vi "Stop.vi"(8 "error in (no error)":errorcluster, 11 "XNET_CAN_RW in":refnum<class "XNET CAN RW.lvclass">) -> (0 "error out":errorcluster, 3 "XNET_CAN_RW out":refnum<class "XNET CAN RW.lvclass">)   [LabVIEW 2021, in "XNET CAN RW.lvclass"]
uses:
  XNET CAN RW.lvclass
  XNET CAN RW.lvclass/XNET CAN RW.ctl
  <vilib>/Utility/error.llb/Clear Errors.vi
  Utilities/Add Error.vi
  <vilib>/xnet/xnet.llb/XNET Wait (Transmit Complete).vi
  Utilities/Add Error Core.vi
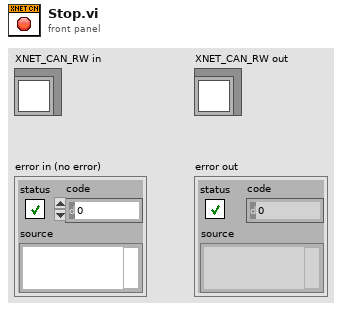
[diagram p1: front panel]
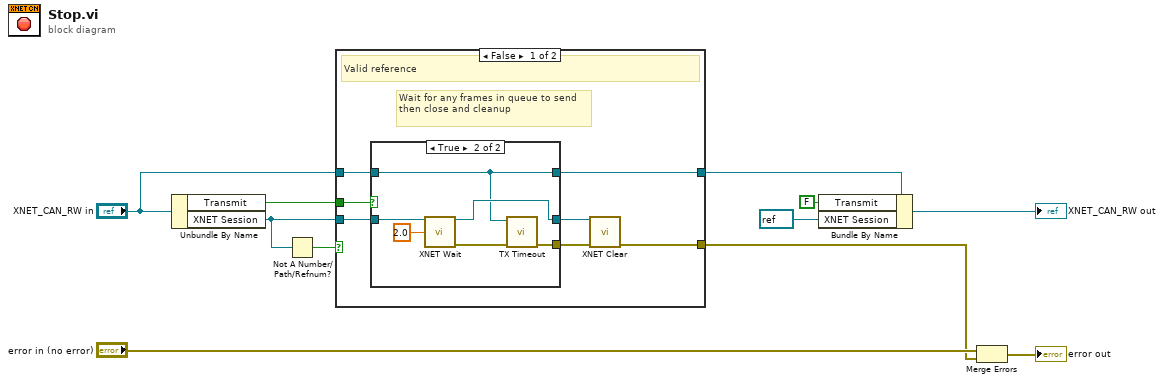
[diagram p0: block diagram]
diagram:
  n1 = Unbundle By Name("XNET_CAN_RW in") -> ("Transmit"=w4:bool, "XNET Session"=w6:refnum<k21>)
  n2 = Not A Number/Path/Refnum?(number/path/refnum=w6) -> (NaN/Path/Refnum?=w7:bool)
  n3 = case shown="False" w7 {
    tunnel: w6 -> [w18 _]
    tunnel: [w17 _] -> w9
    tunnel: w4 -> [w14 _]
    tunnel: "XNET_CAN_RW in" -> [w13 w27]
    tunnel: [w12 w27] -> w1
    frame False {
      # "Wait for any frames in queue to send then close and cleanup"
      # "Valid reference"
      n4 = case shown="True" w14 {
        tunnel: w18 -> [w20 w26]
        tunnel: [w20 w22] -> w16
        tunnel: [_ w24] -> w15
        tunnel: w13 -> [w19 w21]
        tunnel: [w19 w21] -> w12
        frame False {
        }
        frame True {
          n5 = call-poly <vilib>:"XNET Wait.vi"("session in"=w26, "timeout (10)"=2.0) -> ("session out"=w22:refnum<k21>, "error out"=w25:errorcluster)  [unwired: 12 in]
          n6 = call "TX Timeout.vi"("error in (no error)"=w25, "XNET_CAN_RW in"=w21) -> ("error out"=w24:errorcluster)  [unwired: 8 in, 1 out]
        }
      }
      n7 = call <vilib>:"XNET Clear.vi"("session in"=w16, "error in (no error)"=w15) -> ("error out"=w17:errorcluster)  [unwired: 13 in]
    }
    frame True {
      # "Not valid reference"
    }
  }
  n8 = Bundle By Name(cluster=w1, "Transmit"=FALSE, "XNET Session"=refnum<k21> refnum) -> (→"XNET_CAN_RW out":refnum<class "XNET CAN RW.lvclass">)
  n9 = Merge Errors("error in (no error)", w9) -> (→"error out":errorcluster)
